vi "Handle Error.vi"(8 "error in (no error)":errorcluster, 11 "ChannelManagerUI in":refnum<class "ChannelManagerUI.lvclass">) -> (0 "error out":errorcluster, 2 "stop actor?":bool=TRUE, 3 "ChannelManagerUI out":refnum<class "ChannelManagerUI.lvclass">)   [LabVIEW 2021, in "Channel.lvlib" / "ChannelManagerUI.lvlib" / "ChannelManagerUI.lvclass"]
doc: "<p>(<strong>Filename</strong>: <span class=\"dnl\">Actor Framework.lvlib:Actor.lvclass:Handle Error.vi</span>)</p>\n<p>Defines how the actor handles an error that occurred while processing a message. By default, this method does nothing except stop the actor.</p>"
uses:
  ChannelManagerUI.lvclass
  ChannelsManager/ChannelsManager/ChannelsManager.lvclass
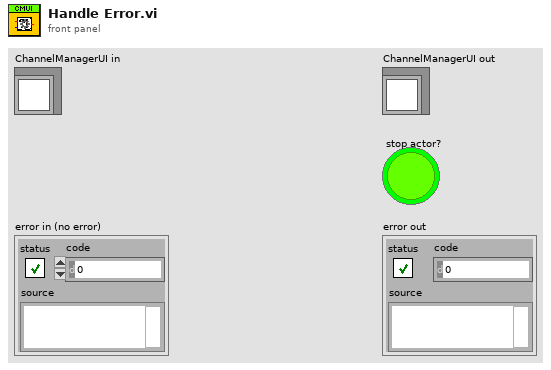
[diagram p1: front panel]
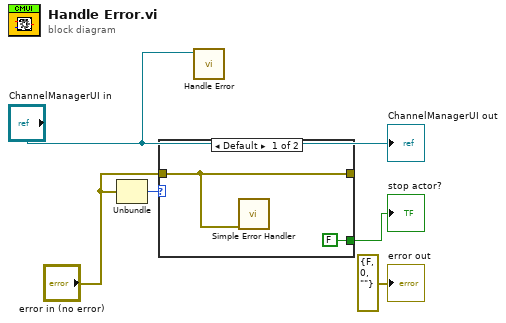
[diagram p0: block diagram]
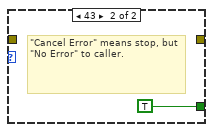
[diagram p2: hidden frame]
diagram:
  n1 = Unbundle("error in (no error)") -> ("code"=w5:i32)  [unwired: 2 out]
  n2 = case shown="Default" w5 {
    tunnel: [w6 _] -> _
    tunnel: "error in (no error)" -> [w6 _]
    tunnel: [FALSE ("stop actor?") TRUE ("stop actor?")] -> w3
    frame Default {
      n3 = call <vilib>:"Simple Error Handler.vi"("error in (no error)"=w6) -> ()  [unwired: 4 in, 5 out]
    }
    frame 43 {
      # "\"Cancel Error\" means stop, but \"No Error\" to caller."
    }
  }
  "stop actor?" <- w3
  n4 = call-parent "Handle Error.vi"("Actor in"="ChannelManagerUI in") -> ()  [unwired: 8 in, 3 out]
  "ChannelManagerUI out" <- "ChannelManagerUI in"
  "error out" <- errorcluster {"status"=FALSE, "code"=0, "source"=""} ("error out")
